vi "Set User FullName.vi"(5 "Save File":bool=TRUE, 6 "error in (no error)":errorcluster, 7 "FullName":string, 8 "LoginName":string, 9 "EasyUserManager in":refnum<class "EasyUserManager.lvclass">) -> (0 "error out":errorcluster, 3 "EasyUserManager out":refnum<class "EasyUserManager.lvclass">)   [LabVIEW 2024, in "EasyUserManager.lvclass"]
doc: "Set <B>FullName</B> of the user specified by <B>LoginName</B>. \n\nThe boolean input <B>Save File</B> controls whether changes are immediately saved to the users file (Default: True)."
uses:
  EasyUserManager.lvclass
  EasyUserManager.lvclass/EasyUserManager.ctl
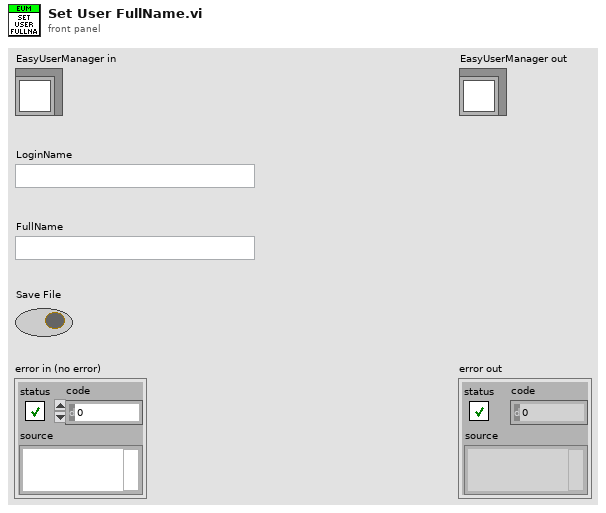
[diagram p1: front panel]
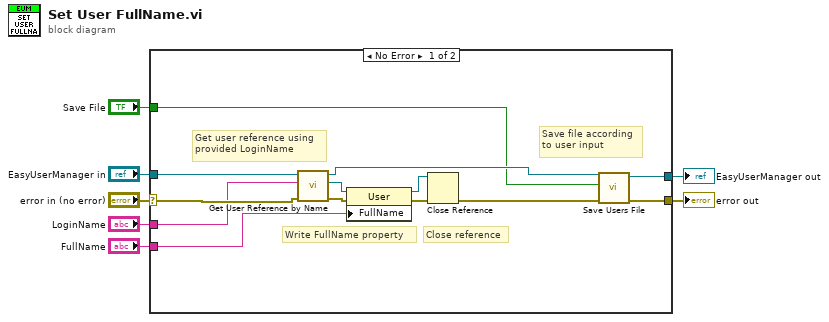
[diagram p0: block diagram]
diagram:
  n1 = case shown="No Error" "error in (no error)" {
    selector: "error in (no error)" -> [w11 w22]
    tunnel: [w12 w22] -> w6
    tunnel: [w14 w21] -> w4
    tunnel: "EasyUserManager in" -> [w20 w21]
    tunnel: "LoginName" -> [w10 _]
    tunnel: "FullName" -> [w9 _]
    tunnel: "Save File" -> [w8 _]
    frame No Error {
      # "Close reference"
      # "Write FullName property"
      # "Get user reference using \nprovided LoginName"
      # "Save file according\nto user input"
      n2 = call "Get User Reference by Name.vi"("error in (no error)"=w11, "LoginName"=w10, "EasyUserManager in"=w20) -> ("error out"=w18:errorcluster, "User Reference"=w19:refnum<k7>, "EasyUserManager out"=w15:refnum<class "EasyUserManager.lvclass">)  [unwired: 2 in]
      n3 = property on="Property Node" class="User"(reference=w19, error in=w18, "FullName"=w9) -> (reference out=w17:refnum<k7>, error out=w16:errorcluster)
      n4 = Close Reference(reference=w17, error in (no error)=w16) -> (error out=w13:errorcluster)
      n5 = call "Save Users File.vi"("error in (no error)"=w13, "Save"=w8, "EasyUserManager in"=w15) -> ("error out"=w12:errorcluster, "EasyUserManager out"=w14:refnum<class "EasyUserManager.lvclass">)  [unwired: 3 in]
    }
    frame Error {
      # "Pass error and do nothing."
    }
  }
  "error out" <- w6
  "EasyUserManager out" <- w4
